vi "Ex seqlist.vi"() -> (0 "S array":T1(array[cluster]), 2 "selected Seq":string[](array[string]), 3 "selected sample name":string[](array[string]))   [LabVIEW 2018]
panel:
  in  "path":string="005.csv"
  in  "Select Base list":bool
  in  "All_Select":bool
  in  "Seqlist Renew":bool
  in  "Save":bool
  in  "load":bool
  out "size(s)":i32
  in  "Cluster":T2={"Right Read MIN"=6, "STD Type"=enum."Region", "Selection"=enum."10kHz", "Filter P"=0, "noise MAX"=3}
  out "S New Info and MiN out":T3={"Sample Sequence"="GATGATGATGATGATGAT", "Right Read MIN"=6, "Filter P"=0, "STD Type"=enum."Region", "Base Table"=[], "Selection"=enum."10kHz", "noise MAX"=3, "Sample name"=""} {"Base Table"."Value 3" format="%.2g"}
  out "Base Table":T4(array[cluster]) {"Value 3" format="%.2g"}
  out "Seq":string[](array[string])
  in  "EX":string[](array[string])
  out "All Ready?":bool
  in  "All_Clear":bool
  in  "Delete":bool
  out "F_Array":cluster{string, bool}[](array[cluster])
  out "Ready!":bool
  out "sorted array":string[](array[string])
  out "path 2":path
  out "SX#":i32
  out "location":string
  out "PC":string
  out "sample name":string[](array[string])
  in  "Go Net":bool
  in  "Scrollbar V 2":i32(c297)
  out "error out":errorcluster
  in  "error in":errorcluster
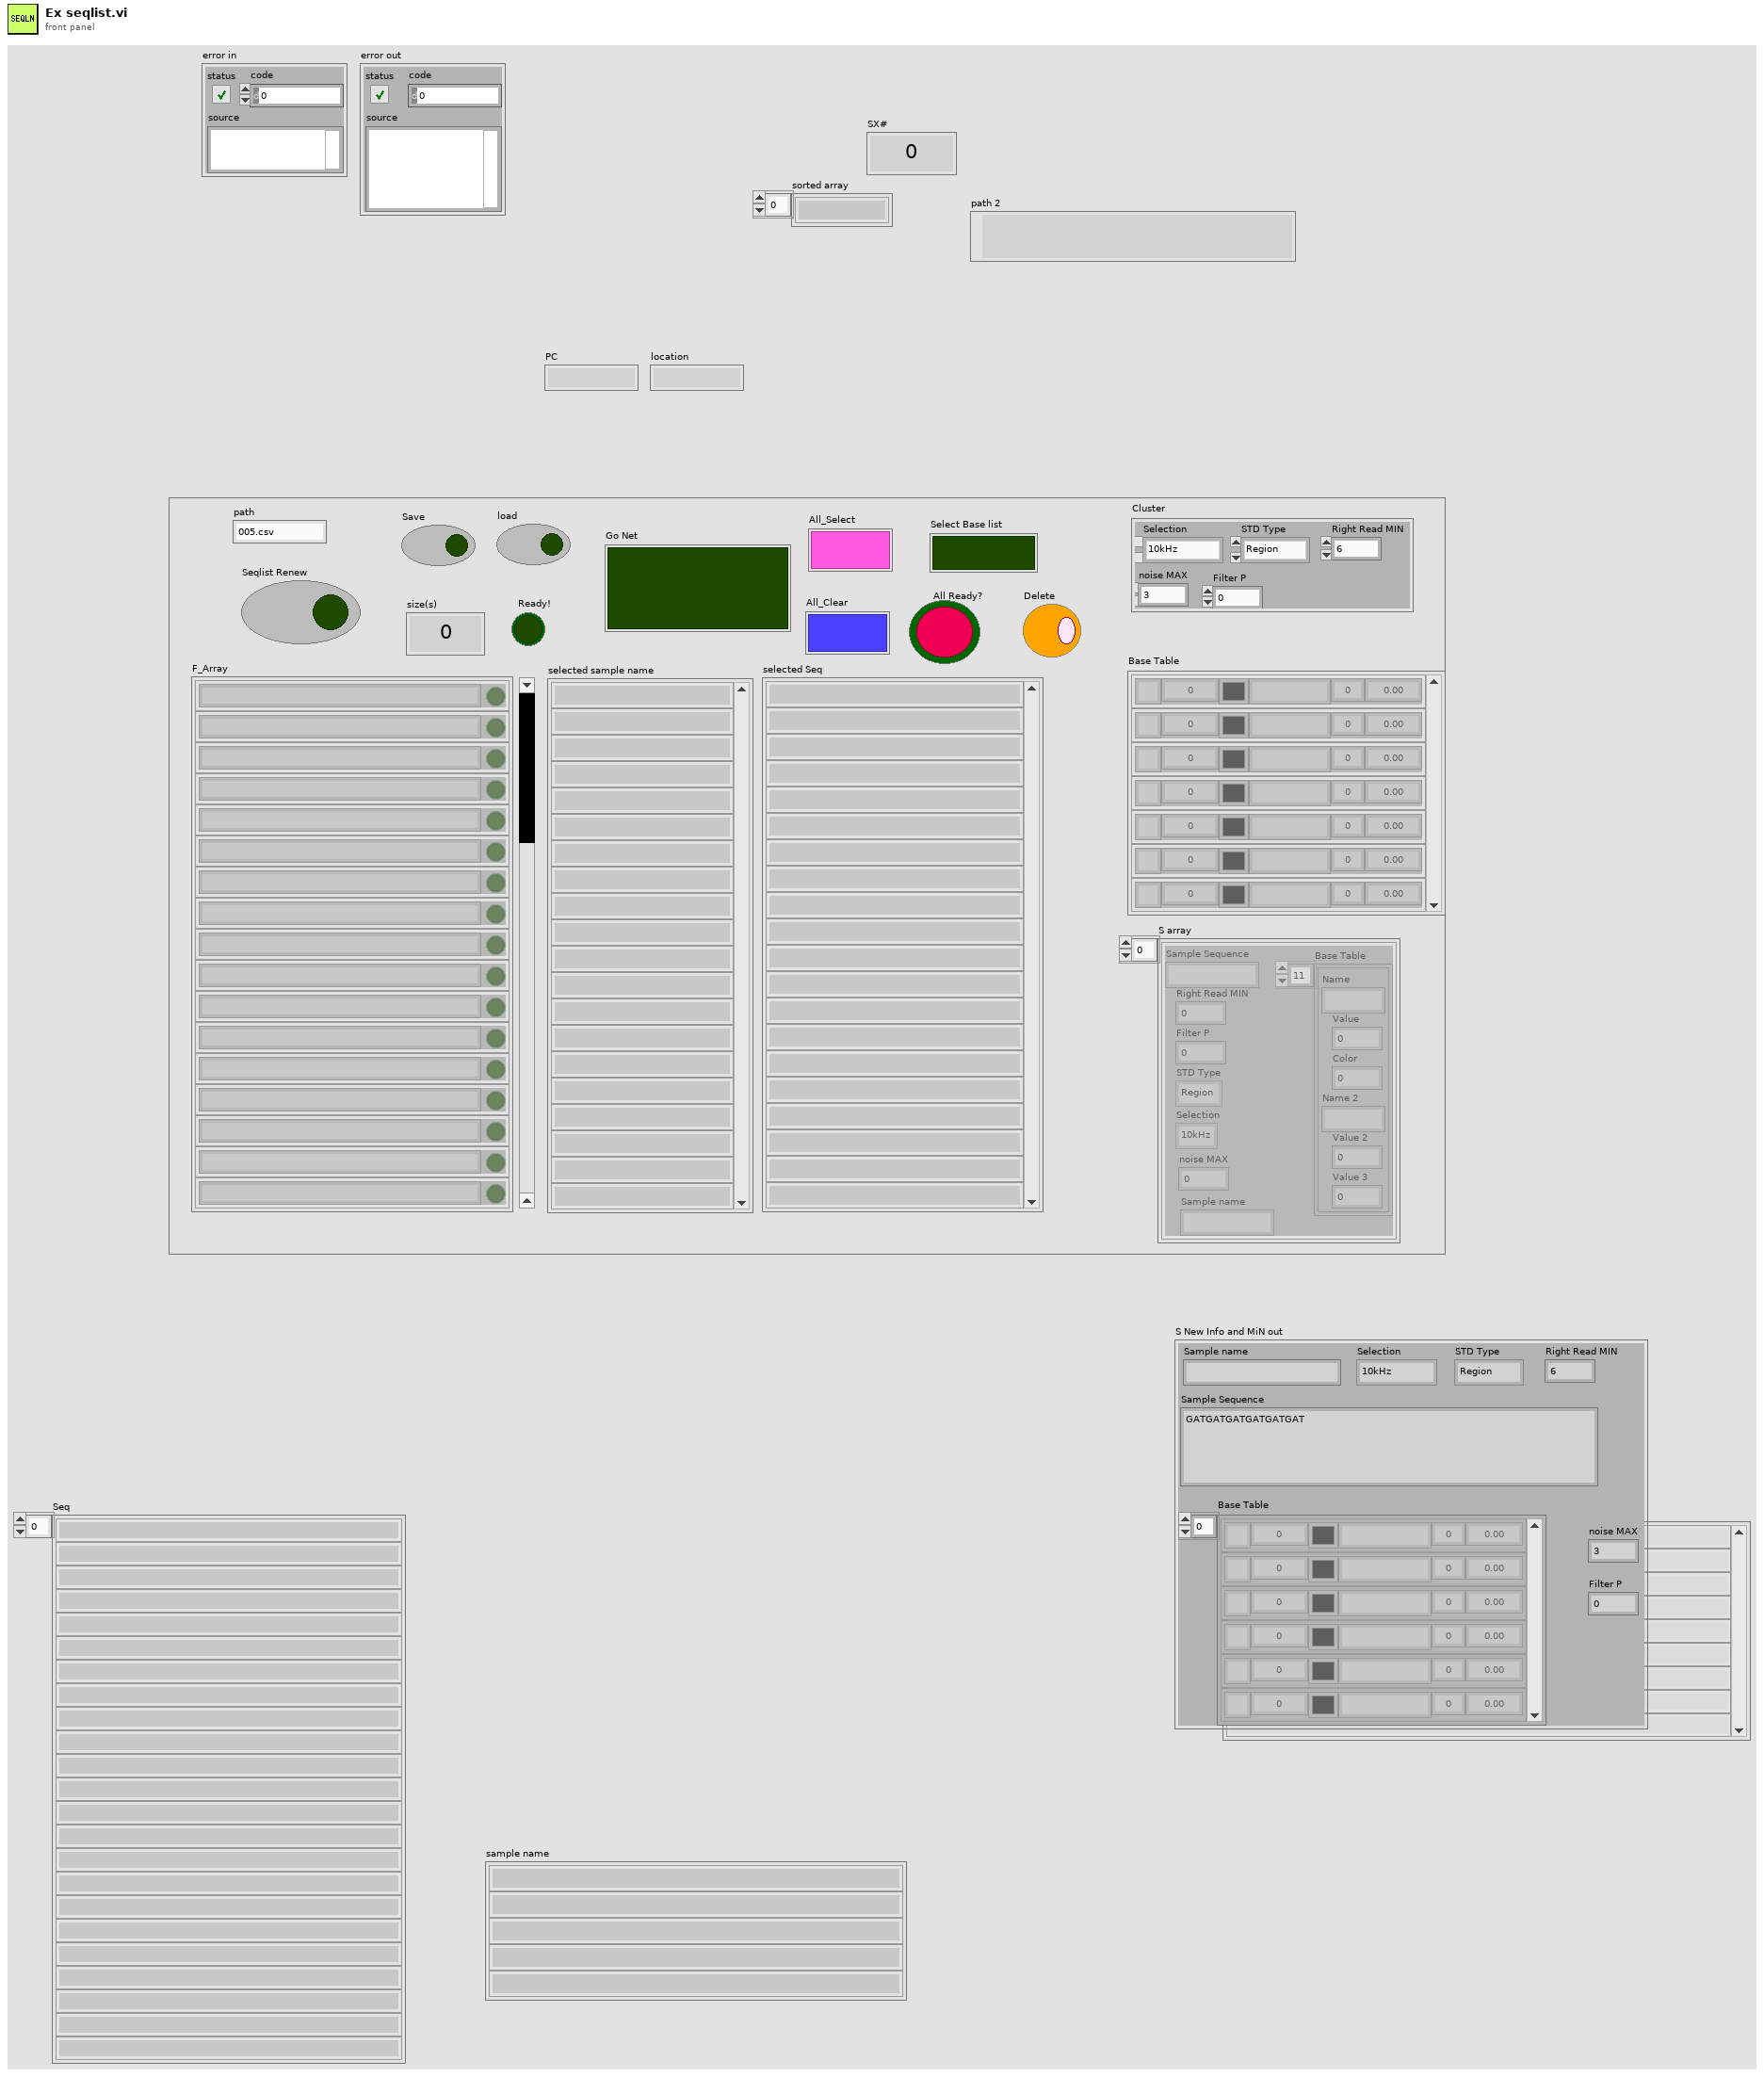
[diagram p1: front panel]
types:
  T1 = cluster{"Sample Sequence":string, "Right Read MIN":i32, "Filter P":i32, "STD Type":enum16{"Region", "Each", "Fixed"}, "Base Table":cluster{"Name":string, "Value":dbl, "Color":u32, "Name 2":string, "Value 2":dbl, "Value 3":dbl}[], "Selection":enum16{"10kHz", "100kHz"}, "noise MAX":i32, "Sample name":string}[]
  T2 = cluster{"Right Read MIN":i32, "STD Type":enum16{"Region", "Each", "Fixed"}, "Selection":enum16{"10kHz", "100kHz"}, "Filter P":i32, "noise MAX":i32}
  T3 = cluster{"Sample Sequence":string, "Right Read MIN":i32, "Filter P":i32, "STD Type":enum16{"Region", "Each", "Fixed"}, "Base Table":cluster{"Name":string, "Value":dbl, "Color":u32, "Name 2":string, "Value 2":dbl, "Value 3":dbl}[], "Selection":enum16{"10kHz", "100kHz"}, "noise MAX":i32, "Sample name":string}
  T4 = cluster{"Name":string, "Value":dbl, "Color":u32, "Name 2":string, "Value 2":dbl, "Value 3":dbl}[]
  T5 = cluster{"Sample ID":string, "Right Read MIN":i32, "Filter P":i32, "STD Type":enum16{"Region", "Each", "Fixed"}, "Base All Composition":cluster{"Name":string, "Value":dbl, "Color":u32, "Name 2":string, "Value 2":dbl, "Value 3":dbl}[], "Selection":enum16{"10kHz", "100kHz"}, "noise MAX":i32, string}[]
  T6 = typedef "LVPoint32TypeDef.ctl" = cluster{"Horizontal":i32, "Vertical":i32}
  T7 = typedef "LVPositionTypeDef.ctl" = cluster{"Left":i32, "Top":i32}
  T8 = typedef "LVBoundsTypeDef.ctl" = cluster{"Width":u32, "Height":u32}
  T9 = cluster{"Sample ID":string, "Right Read MIN":i32, "Filter P":i32, "STD Type":enum16{"Region", "Each", "Fixed"}, "Base All Composition":cluster{"Name":string, "Value":dbl, "Color":u32, "Name 2":string, "Value 2":dbl, "Value 3":dbl}[], "Selection":enum16{"10kHz", "100kHz"}, "noise MAX":i32, string}
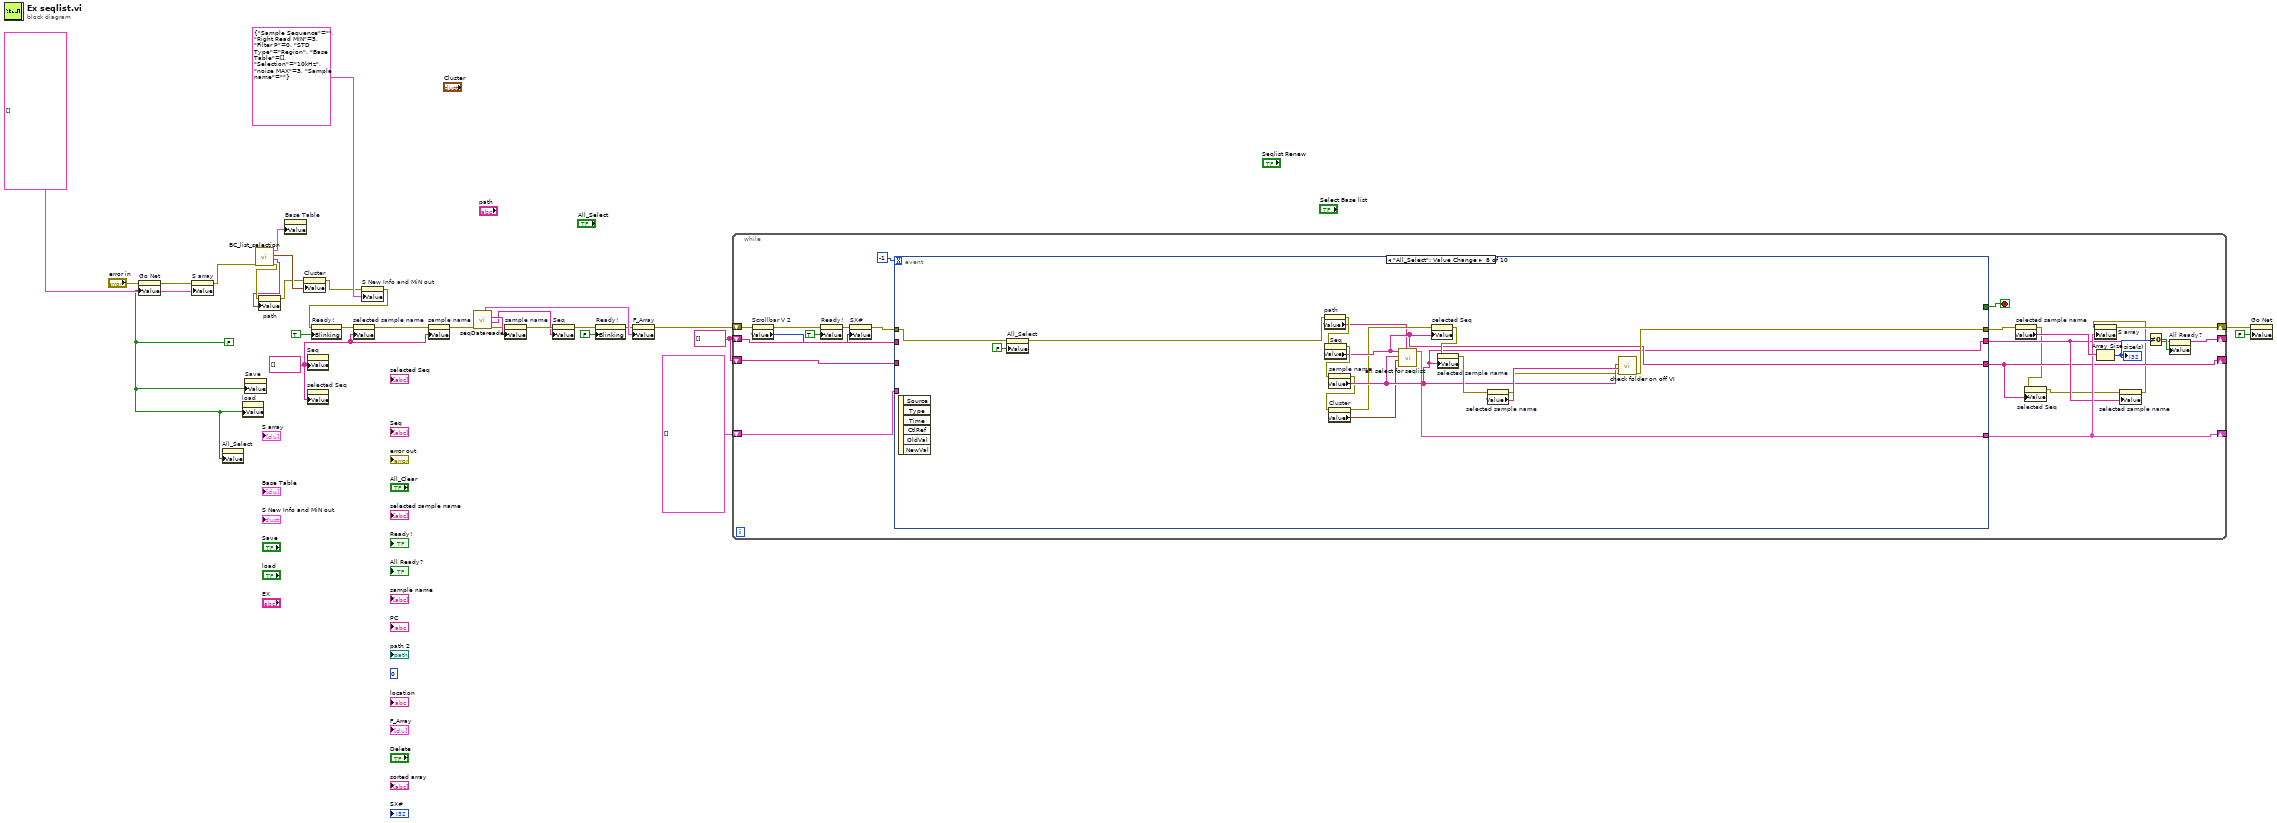
[diagram p0: block diagram]
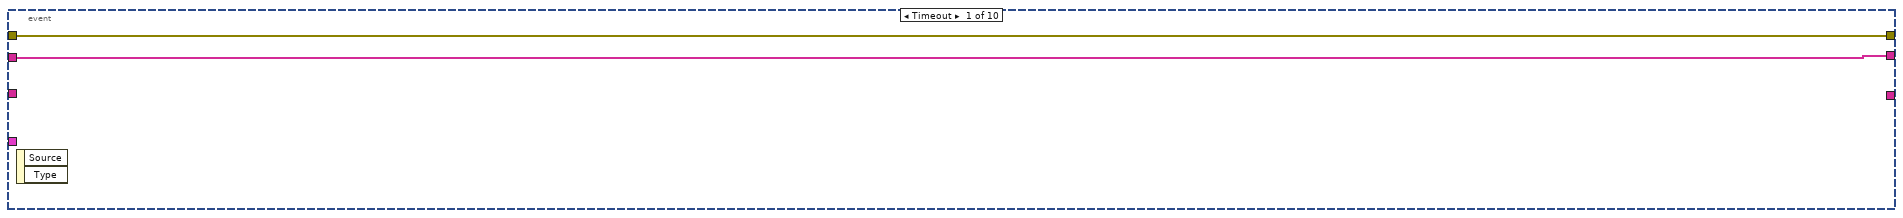
[diagram p2: hidden frame]
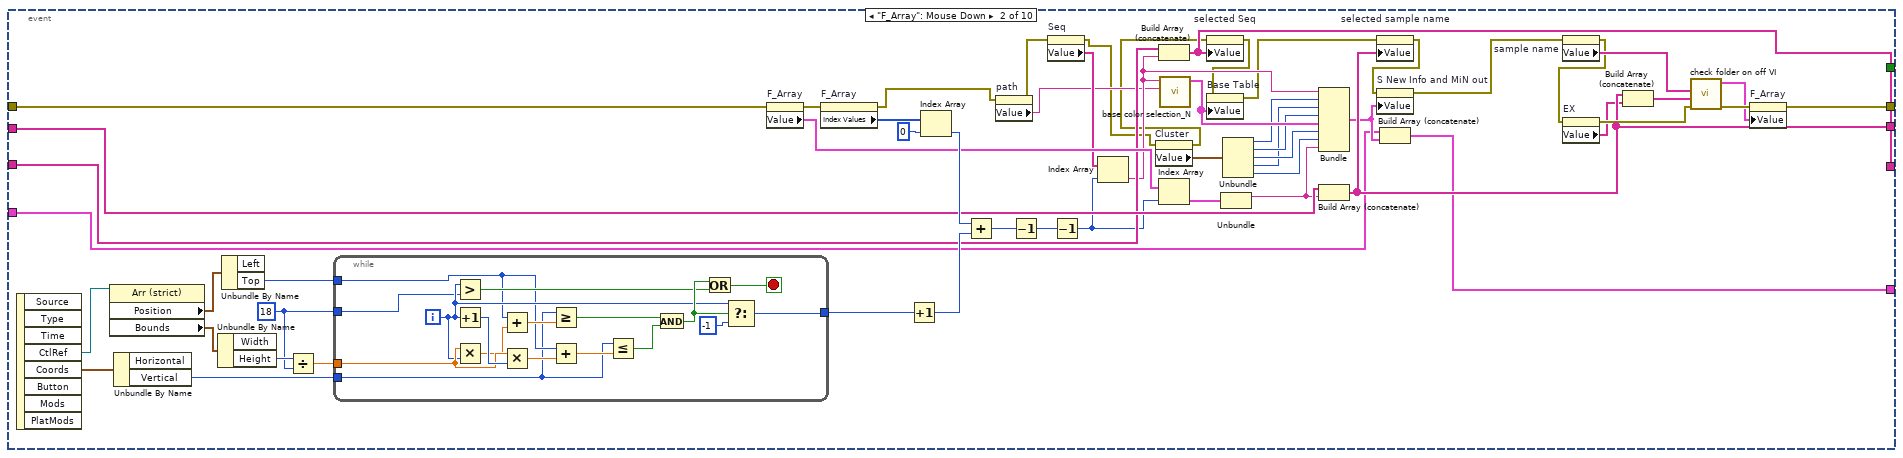
[diagram p3: hidden frame]
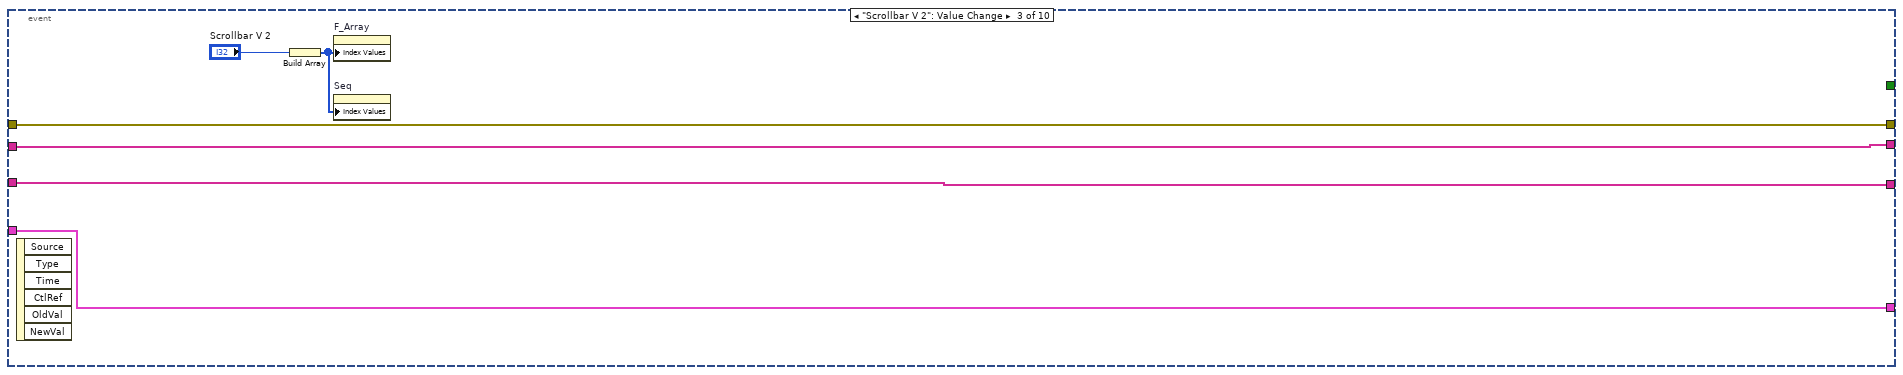
[diagram p4: hidden frame]
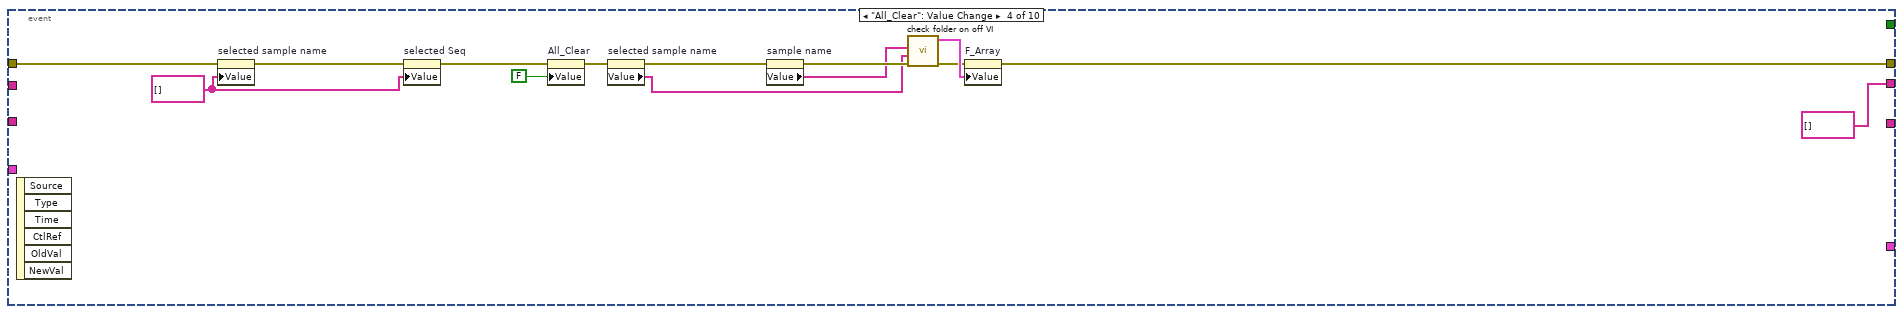
[diagram p5: hidden frame]
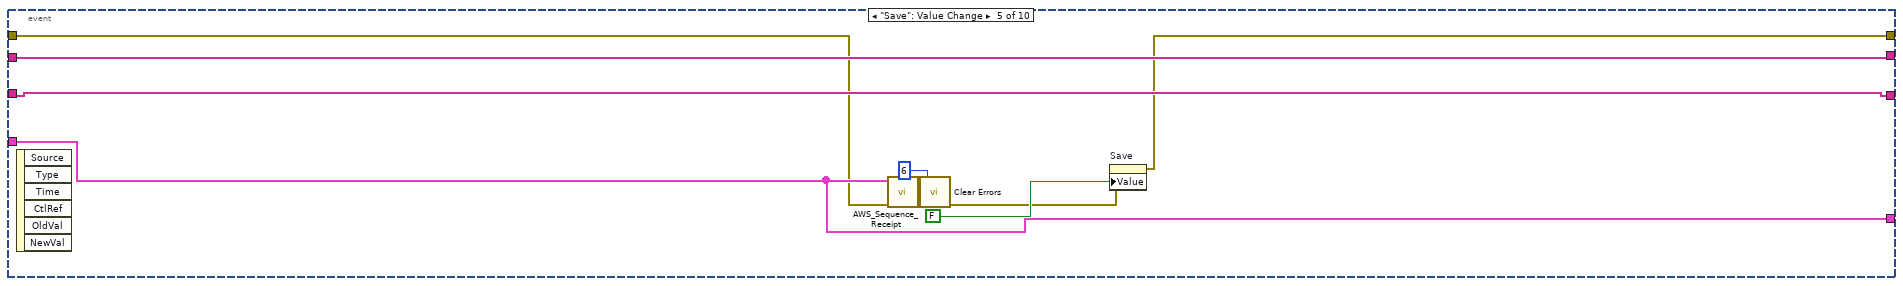
[diagram p6: hidden frame]
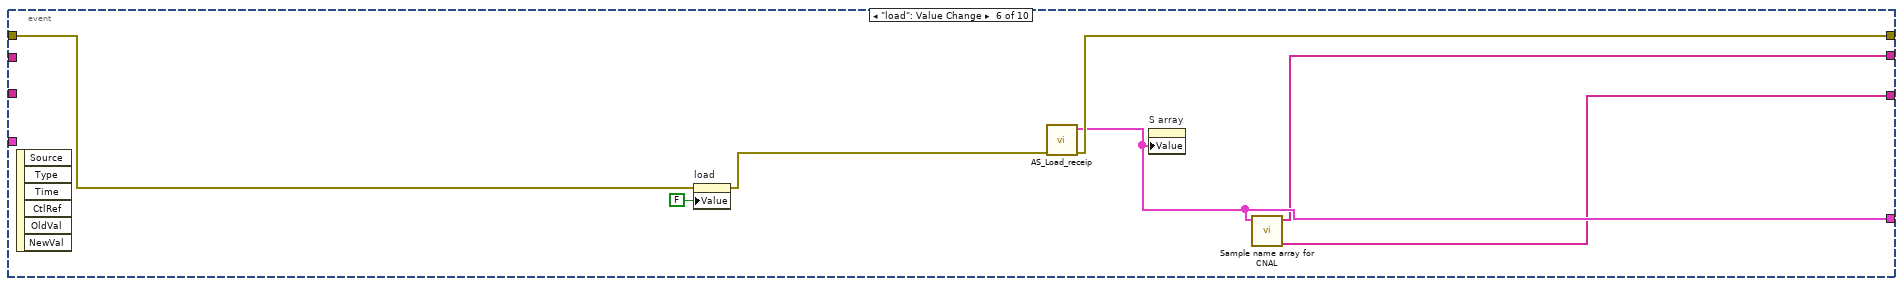
[diagram p7: hidden frame]
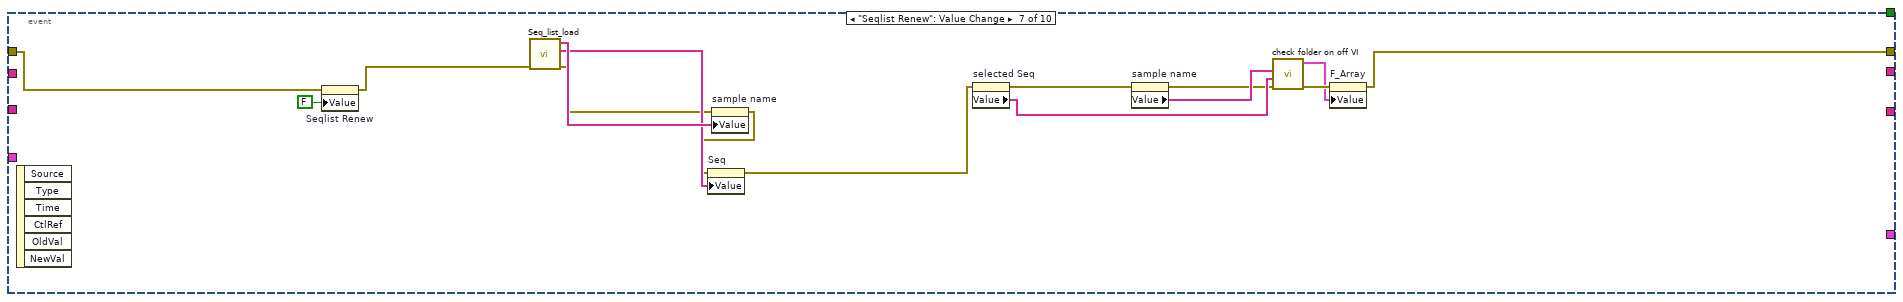
[diagram p8: hidden frame]
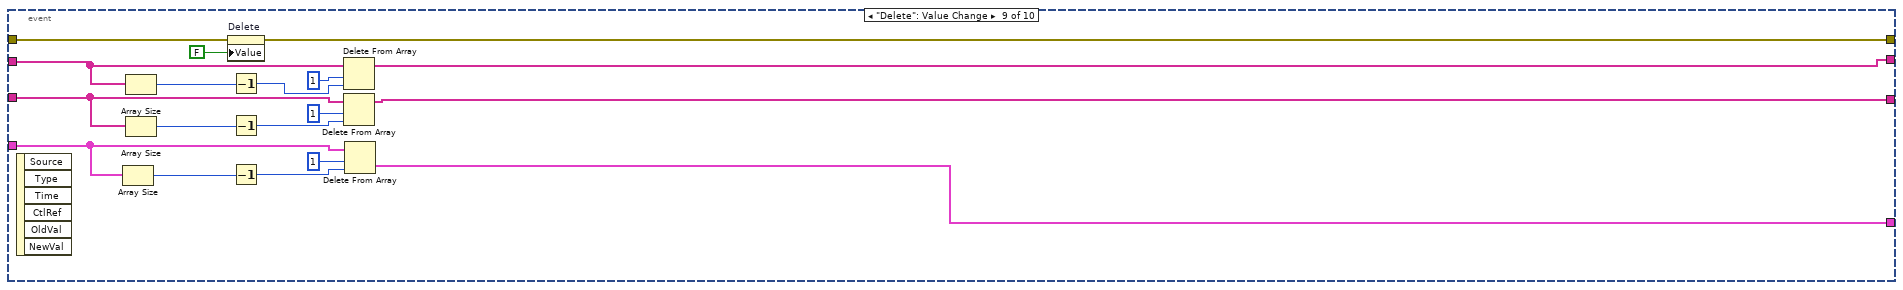
[diagram p9: hidden frame]
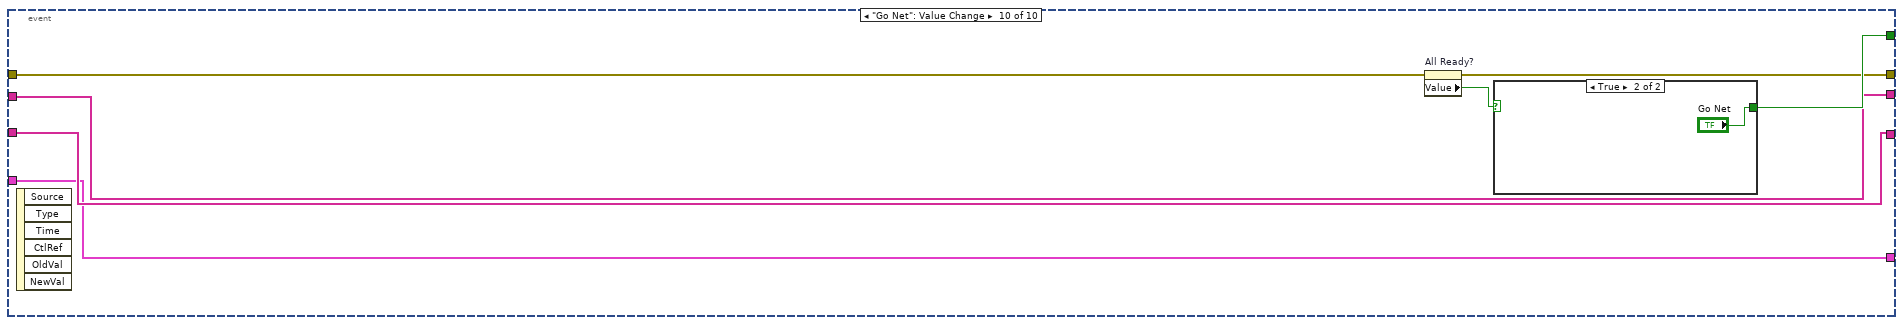
[diagram p10: hidden frame]
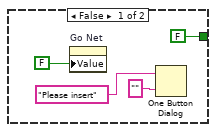
[diagram p11: hidden frame]
diagram:
  (unwired) 0 ("EX_IDX")
  w15 = string[] []
  w16 = string[] []
  w8 = FALSE ("10kHz_upload")
  n1 = property on="Go Net" class="Bool (strict)"(error in="error in", "Value"=w8) -> (error out=w11:errorcluster)  [unwired: 1 in, 1 out]
  n2 = property on="S array" class="Arr (strict)"(error in=w11, "Value"=T1 [] ("S array 2")) -> (error out=w5:errorcluster)  [unwired: 1 in, 1 out]
  n3 = property on="All_Select" class="Bool (strict)"("Value"=w8) -> ()  [unwired: 2 in, 2 out]
  n4 = property on="load" class="Bool (strict)"("Value"=w8) -> ()  [unwired: 2 in, 2 out]
  n5 = property on="Save" class="Bool (strict)"("Value"=w8) -> ()  [unwired: 2 in, 2 out]
  n6 = call "BC_list_selection.vi"("error in"=w5) -> ("error out"=w4:errorcluster, "path"=w2:string, "Cluster"=w6:T2, "Base All Composition"=w1:T4)  [unwired: 7 in]
  n7 = property on="path" class="Str"(error in=w4, "Value"=w2) -> (error out=w3:errorcluster)  [unwired: 1 in, 1 out]
  n8 = property on="Base Table" class="Arr (strict)"("Value"=w1) -> ()  [unwired: 2 in, 2 out]
  n9 = property on="Cluster" class="Clust (strict)"(error in=w3, "Value"=w6) -> (error out=w7:errorcluster)  [unwired: 1 in, 1 out]
  n10 = property on="Seq" class="Arr (strict)"("Value"=w15) -> ()  [unwired: 2 in, 2 out]
  n11 = property on="selected Seq" class="Arr (strict)"("Value"=w15) -> ()  [unwired: 2 in, 2 out]
  n12 = property on="S New Info and MiN out" class="Clust (strict)"(error in=w7, "Value"=T3 {"Sample Sequence"="", "Right Read MIN"=5, "Filter P"=0, "STD Type"=enum."Region", "Base Table"=[], "Selection"=enum."10kHz", "noise MAX"=3, "Sample name"=""} ("S New Info and MiN out 2")) -> (error out=w9:errorcluster)  [unwired: 1 in, 1 out]
  n13 = property on="Ready!" class="Bool (strict)"(error in=w9, "Blinking"=TRUE) -> (error out=w25:errorcluster)  [unwired: 1 in, 1 out]
  n14 = property on="selected sample name" class="Arr (strict)"(error in=w25, "Value"=w15) -> (error out=w27:errorcluster)  [unwired: 1 in, 1 out]
  n15 = property on="sample name" class="Arr (strict)"(error in=w27, "Value"=w15) -> (error out=w13:errorcluster)  [unwired: 1 in, 1 out]
  n16 = call "seqDatareader.vi"("エラー入力"=w13) -> ("error out"=w21:errorcluster, "Seq"=w17:string[], "Seq_name"=w22:string[], "Array 3"=w24:cluster{string, bool}[])  [unwired: 6 in, 1 out]
  n17 = property on="sample name" class="Arr (strict)"(error in=w21, "Value"=w22) -> (error out=w19:errorcluster)  [unwired: 1 in, 1 out]
  n18 = property on="Seq" class="Arr (strict)"(error in=w19, "Value"=w17) -> (error out=w18:errorcluster)  [unwired: 1 in, 1 out]
  n19 = property on="Ready!" class="Bool (strict)"(error in=w18, "Blinking"=FALSE ("Ready!")) -> (error out=w23:errorcluster)  [unwired: 1 in, 1 out]
  n20 = property on="F_Array" class="Arr (strict)"(error in=w23, "Value"=w24) -> (error out=w28:errorcluster)  [unwired: 1 in, 1 out]
  n21 = while {
    shift-right: [w36] -> _
    shift-left: w16 -> [w51]
    shift-right: [w37] -> w20
    shift-left: w28 -> [w50]
    shift-right: [w35] -> _
    shift-left: w16 -> [w41]
    shift-right: [w39] -> _
    shift-left: T5 [] -> [w40]
    stop <- w52 stop-if-true
    n22 = property on="Scrollbar V 2" class="Scroll (strict)"(error in=w50) -> (error out=w47:errorcluster, "Value"=w49:i32)  [unwired: 1 in, 1 out]
    n23 = property on="Ready!" class="Bool (strict)"(error in=w47, "Value"=TRUE ("Ready!")) -> (error out=w46:errorcluster)  [unwired: 1 in, 1 out]
    n24 = property on="SX#" class="DigNum (strict)"(error in=w46, "Value"=w49) -> (error out=w42:errorcluster)  [unwired: 1 in, 1 out]
    n25 = event shown="[7] \"All_Select\": Value Change" {
      selector: _ -> [_ _ _ _ _ _ _ _ _ _]
      dyn-events: _ -> [_ _ _ _ _ _ _ _ _ _]
      timeout: -1 -> [_ _ _ _ _ _ _ _ _ _]
      tunnel: [w55 w89 w132 w140 w148 w163 w164 w191 w211 w217] -> w44
      tunnel: [w54 w85 w133 string[] [] w151 w161 _ w186 w200 w219] -> w36
      tunnel: w51 -> [w54 w92 w133 _ w151 _ _ _ w198 w219]
      tunnel: [_ _ _ _ _ _ _ _ _ w220] -> w52
      tunnel: w42 -> [w55 w82 w132 w139 w149 w158 w177 w195 w212 w218]
      tunnel: w41 -> [_ w81 w129 _ w150 _ _ _ w196 w215]
      tunnel: [_ w78 w129 _ w150 w160 _ w187 w199 w215] -> w35
      tunnel: [_ w66 w128 _ w152 w162 _ w192 w201 w214] -> w39
      tunnel: w40 -> [_ w67 w128 _ w152 _ _ _ w197 w214]
      event Timeout {
        n26 = event-data() -> ()  [unwired: 1 in, 2 out]
      }
      event "F_Array": Mouse Down {
        w102 = 18 ("f")
        n27 = event-data() -> ("CtlRef"=w94:refnum<vi>, "Coords"=w93:T6)  [unwired: 1 in, 6 out]
        n28 = property class="Arr (strict)"(reference=w94) -> ("Position"=w108:T7, "Bounds"=w107:T8)  [unwired: 1 in, 2 out]
        n29 = Unbundle By Name(w93) -> ("Vertical"=w106:i32)  [unwired: 1 out]
        n30 = Unbundle By Name(w107) -> ("Height"=w105:u32)  [unwired: 1 out]
        n31 = Unbundle By Name(w108) -> ("Top"=w103:i32)  [unwired: 1 out]
        n32 = Divide(x=w105, y=w102) -> (x/y=w104:dbl)
        n33 = while {
          tunnel: w106 -> [w111]
          tunnel: w104 -> [w117]
          tunnel: w103 -> [w113]
          tunnel: [w122] -> w98
          tunnel: w102 -> [w112]
          i -> [w116]
          stop <- w120 stop-if-true
          n34 = Greater?(x=w116, y=w112) -> (0:w118:bool)
          n35 = Increment(x=w116) -> (x+1=w127:i32)
          n36 = Multiply(x=w117, y=w116) -> (x*y=w114:dbl)
          n37 = Add(x=w113, y=w114) -> (x+y=w115:dbl)
          n38 = Multiply(x=w117, y=w127) -> (x*y=w125:dbl)
          n39 = Greater Or Equal?(x=w111, y=w115) -> (x >= y?=w124:bool)
          n40 = Add(x=w113, y=w125) -> (x+y=w126:dbl)
          n41 = Less Or Equal?(x=w111, y=w126) -> (x <= y?=w123:bool)
          n42 = And(x=w124, y=w123) -> (x .and. y?=w119:bool)
          n43 = Or(x=w119, y=w118) -> (x .or. y?=w120:bool)
          n44 = Select(t=w116, s=w119, f=-1) -> (s? t:f=w122:i32)
        }
        n45 = property on="F_Array" class="Arr (strict)"(error in=w82) -> (error out=w96:errorcluster, "Value"=w97:cluster{string, bool}[])  [unwired: 1 in, 1 out]
        n46 = property on="F_Array" class="Arr (strict)"(error in=w96) -> (error out=w62:errorcluster, "Index Values"=w109:u32[])  [unwired: 1 in, 1 out]
        n47 = Increment(x=w98) -> (x+1=w101:i32)
        n48 = Index Array(array=w109, index=0 ("指標")) -> (element=w99:u32)
        n49 = Add(x=w99, y=w101) -> (x+y=w100:u32)
        n50 = property on="path" class="Str"(error in=w62) -> (error out=w61:errorcluster, "Value"=w65:string)  [unwired: 1 in, 1 out]
        n51 = Decrement(x=w100) -> (x-1=w95:u32)
        n52 = property on="Seq" class="Arr (strict)"(error in=w61) -> (error out=w64:errorcluster, "Value"=w80:string[])  [unwired: 1 in, 1 out]
        n53 = Decrement(x=w95) -> (x-1=w79:u32)
        n54 = Index Array(array=w80, index=w79) -> (element=w75:string)
        n55 = property on="Cluster" class="Clust (strict)"(error in=w64) -> (error out=w63:errorcluster, "Value"=w74:T2)  [unwired: 1 in, 1 out]
        n56 = Build Array (concatenate)(w81, w75) -> (w78:string[])
        n57 = Index Array(array=w97, index=w79) -> (element=w91:cluster{string, bool})
        n58 = call "base color selection_N.vi"("path"=w65, "Sample Sequence"=w75) -> ("Base All Composition"=w77:T4)  [unwired: 8 in, 1 out]
        n59 = property on="selected Seq" class="Arr (strict)"(error in=w63, "Value"=w78) -> (error out=w60:errorcluster)  [unwired: 1 in, 1 out]
        n60 = property on="Base Table" class="Arr (strict)"(error in=w60, "Value"=w77) -> (error out=w59:errorcluster)  [unwired: 1 in, 1 out]
        n61 = Unbundle(w91) -> (w76:string)  [unwired: 1 out]
        n62 = Unbundle(w74) -> ("Right Read MIN"=w73:i32, "STD Type"=w72:enum16{"Region", "Each", "Fixed"}, "Selection"=w71:enum16{"10kHz", "100kHz"}, "Filter P"=w69:i32, "noise MAX"=w70:i32)
        n63 = Bundle("Sample ID"=w75, "Right Read MIN"=w73, "Filter P"=w69, "STD Type"=w72, "Base All Composition"=w77, "Selection"=w71, "noise MAX"=w70, w76) -> (w68:T9)  [unwired: 1 in]
        n64 = Build Array (concatenate)(w92, w76) -> (w85:string[])
        n65 = property on="selected sample name" class="Arr (strict)"(error in=w59, "Value"=w85) -> (error out=w58:errorcluster)  [unwired: 1 in, 1 out]
        n66 = property on="S New Info and MiN out" class="Clust (strict)"(error in=w58, "Value"=w68) -> (error out=w57:errorcluster)  [unwired: 1 in, 1 out]
        n67 = Build Array (concatenate)(w67, w68) -> (w66:T5)
        n68 = property on="sample name" class="Arr (strict)"(error in=w57) -> (error out=w56:errorcluster, "Value"=w86:string[])  [unwired: 1 in, 1 out]
        n69 = property on="EX" class="Arr (strict)"(error in=w56) -> (error out=w87:errorcluster, "Value"=w84:string[])  [unwired: 1 in, 1 out]
        n70 = Build Array (concatenate)(w85, w84) -> (w83:string[])
        n71 = call "check folder on off VI.vi"("エラー入力"=w87, "selected EX"=w83, "folder names"=w86) -> ("error out"=w90:errorcluster, "Array 3"=w88:cluster{string, bool}[])  [unwired: 6 in, 1 out]
        n72 = property on="F_Array" class="Arr (strict)"(error in=w90, "Value"=w88) -> (error out=w89:errorcluster)  [unwired: 1 in, 1 out]
      }
      event "Scrollbar V 2": Value Change {
        n73 = event-data() -> ()  [unwired: 1 in, 6 out]
        n74 = Build Array("Scrollbar V 2") -> (w130:i32[])
        n75 = property on="F_Array" class="Arr (strict)"("Index Values"=w130) -> ()  [unwired: 2 in, 2 out]
        n76 = property on="Seq" class="Arr (strict)"("Index Values"=w130) -> ()  [unwired: 2 in, 2 out]
      }
      event "All_Clear": Value Change {
        w136 = string[] []
        n77 = event-data() -> ()  [unwired: 1 in, 6 out]
        n78 = property on="selected sample name" class="Arr (strict)"(error in=w139, "Value"=w136) -> (error out=w135:errorcluster)  [unwired: 1 in, 1 out]
        n79 = property on="selected Seq" class="Arr (strict)"(error in=w135, "Value"=w136) -> (error out=w134:errorcluster)  [unwired: 1 in, 1 out]
        n80 = property on="All_Clear" class="Bool (strict)"(error in=w134, "Value"=FALSE ("All_Clear")) -> (error out=w138:errorcluster)  [unwired: 1 in, 1 out]
        n81 = property on="selected sample name" class="Arr (strict)"(error in=w138) -> (error out=w137:errorcluster, "Value"=w143:string[])  [unwired: 1 in, 1 out]
        n82 = property on="sample name" class="Arr (strict)"(error in=w137) -> (error out=w145:errorcluster, "Value"=w144:string[])  [unwired: 1 in, 1 out]
        n83 = call "check folder on off VI.vi"("エラー入力"=w145, "selected EX"=w143, "folder names"=w144) -> ("error out"=w141:errorcluster, "Array 3"=w142:cluster{string, bool}[])  [unwired: 6 in, 1 out]
        n84 = property on="F_Array" class="Arr (strict)"(error in=w141, "Value"=w142) -> (error out=w140:errorcluster)  [unwired: 1 in, 1 out]
      }
      event "Save": Value Change {
        n85 = event-data() -> ()  [unwired: 1 in, 6 out]
        n86 = call "AWS_Sequence_Receipt.vi"("error in"=w149, "S array"=w152) -> ("error out"=w156:errorcluster)  [unwired: 7 in, 2 out]
        n87 = call <vilib>:"Clear Errors.vi"("error in (no error)"=w156, "specific error code to clear (0: all)"=6) -> ("error out"=w154:errorcluster)  [unwired: 4 in, 1 out]
        n88 = property on="Save" class="Bool (strict)"(error in=w154, "Value"=FALSE ("Save")) -> (error out=w148:errorcluster)  [unwired: 1 in, 1 out]
      }
      event "load": Value Change {
        n89 = event-data() -> ()  [unwired: 1 in, 6 out]
        n90 = property on="load" class="Bool (strict)"(error in=w158, "Value"=FALSE ("load")) -> (error out=w157:errorcluster)  [unwired: 1 in, 1 out]
        n91 = call "AS_Load_receip.vi"("error in"=w157) -> ("error out"=w163:errorcluster, "S array"=w162:T1)  [unwired: 9 in]
        n92 = property on="S array" class="Arr (strict)"("Value"=w162) -> ()  [unwired: 2 in, 2 out]
        n93 = call "Sample name array for CNAL.vi"("S array"=w162) -> ("Sample Sequence array"=w160:string[], "Sample name array"=w161:string[])  [unwired: 9 in]
      }
      event "Seqlist Renew": Value Change {
        n94 = event-data() -> ()  [unwired: 1 in, 6 out]
        n95 = property on="Seqlist Renew" class="Bool (strict)"(error in=w177, "Value"=FALSE ("Seqlist Renew")) -> (error out=w176:errorcluster)  [unwired: 1 in, 1 out]
        n96 = call "Seq_list_load.vi"("error in"=w176) -> ("error out"=w167:errorcluster, "selected Seq"=w168:string[], "selected sample name"=w169:string[])  [unwired: 8 in]
        n97 = property on="sample name" class="Arr (strict)"(error in=w167, "Value"=w169) -> (error out=w166:errorcluster)  [unwired: 1 in, 1 out]
        n98 = property on="Seq" class="Arr (strict)"(error in=w166, "Value"=w168) -> (error out=w165:errorcluster)  [unwired: 1 in, 1 out]
        n99 = property on="selected Seq" class="Arr (strict)"(error in=w165) -> (error out=w175:errorcluster, "Value"=w172:string[])  [unwired: 1 in, 1 out]
        n100 = property on="sample name" class="Arr (strict)"(error in=w175) -> (error out=w170:errorcluster, "Value"=w171:string[])  [unwired: 1 in, 1 out]
        n101 = call "check folder on off VI.vi"("エラー入力"=w170, "selected EX"=w172, "folder names"=w171) -> ("error out"=w174:errorcluster, "Array 3"=w173:cluster{string, bool}[])  [unwired: 6 in, 1 out]
        n102 = property on="F_Array" class="Arr (strict)"(error in=w174, "Value"=w173) -> (error out=w164:errorcluster)  [unwired: 1 in, 1 out]
      }
      event "All_Select": Value Change {
        n103 = event-data() -> ()  [unwired: 1 in, 6 out]
        n104 = property on="All_Select" class="Bool (strict)"(error in=w195, "Value"=FALSE ("All_Select")) -> (error out=w181:errorcluster)  [unwired: 1 in, 1 out]
        n105 = property on="path" class="Str"(error in=w181) -> (error out=w180:errorcluster, "Value"=w179:string)  [unwired: 1 in, 1 out]
        n106 = property on="Seq" class="Arr (strict)"(error in=w180) -> (error out=w193:errorcluster, "Value"=w187:string[])  [unwired: 1 in, 1 out]
        n107 = property on="sample name" class="Arr (strict)"(error in=w193) -> (error out=w184:errorcluster, "Value"=w186:string[])  [unwired: 1 in, 1 out]
        n108 = property on="Cluster" class="Clust (strict)"(error in=w184) -> (error out=w183:errorcluster, "Value"=w182:T2)  [unwired: 1 in, 1 out]
        n109 = call "all select for seqlist.vi"("path"=w179, "Cluster"=w182, "sample name"=w186, "Seq"=w187) -> ("S array"=w192:T1)  [unwired: 7 in]
        n110 = property on="selected Seq" class="Arr (strict)"(error in=w183, "Value"=w187) -> (error out=w189:errorcluster)  [unwired: 1 in, 1 out]
        n111 = property on="selected sample name" class="Arr (strict)"(error in=w189, "Value"=w186) -> (error out=w188:errorcluster)  [unwired: 1 in, 1 out]
        n112 = property on="selected sample name" class="Arr (strict)"(error in=w188) -> (error out=w185:errorcluster, "Value"=w190:string[])  [unwired: 1 in, 1 out]
        n113 = call "check folder on off VI.vi"("エラー入力"=w185, "selected EX"=w190, "folder names"=w186) -> ("error out"=w191:errorcluster)  [unwired: 6 in, 2 out]
      }
      event "Delete": Value Change {
        n114 = event-data() -> ()  [unwired: 1 in, 6 out]
        n115 = Array Size(array=w197) -> (size(s)=w203:i32)
        n116 = Array Size(array=w198) -> (size(s)=w206:i32)
        n117 = Array Size(array=w196) -> (size(s)=w209:i32)
        n118 = property on="Delete" class="Bool (strict)"(error in=w212, "Value"=FALSE ("DF_enter")) -> (error out=w211:errorcluster)  [unwired: 1 in, 1 out]
        n119 = Decrement(x=w206) -> (x-1=w205:i32)
        n120 = Decrement(x=w209) -> (x-1=w208:i32)
        n121 = Decrement(x=w203) -> (x-1=w202:i32)
        n122 = Delete From Array(array=w198, length=1 ("長さ"), index=w205) -> (array with subset deleted=w200:string[])  [unwired: 1 out]
        n123 = Delete From Array(array=w196, length=1 ("長さ"), index=w208) -> (array with subset deleted=w199:string[])  [unwired: 1 out]
        n124 = Delete From Array(array=w197, length=1 ("長さ"), index=w202) -> (deleted portion=w201:T5)  [unwired: 1 out]
      }
      event "Go Net": Value Change {
        n125 = event-data() -> ()  [unwired: 1 in, 6 out]
        n126 = property on="All Ready?" class="Bool (strict)"(error in=w218) -> (error out=w217:errorcluster, "Value"=w216:bool)  [unwired: 1 in, 1 out]
        n127 = case shown="True" w216 {
          tunnel: [FALSE ("END") "Go Net"] -> w220
          frame False {
            n128 = property on="Go Net" class="Bool (strict)"("Value"=FALSE ("All Ready?")) -> ()  [unwired: 2 in, 2 out]
            n129 = One Button Dialog(message="Please insert", button name ("OK")="") -> ()  [unwired: 1 out]
          }
          frame True {
          }
        }
      }
    }
    n130 = property on="selected sample name" class="Arr (strict)"(error in=w44) -> (error out=w34:errorcluster, "Value"=w45:string[])  [unwired: 1 in, 1 out]
    n131 = property on="selected Seq" class="Arr (strict)"(error in=w34, "Value"=w35) -> (error out=w33:errorcluster)  [unwired: 1 in, 1 out]
    n132 = Array Size(array=w45) -> (size(s)=w43:i32)
    "size(s)" <- w43
    n133 = property on="selected sample name" class="Arr (strict)"(error in=w33, "Value"=w36) -> (error out=w32:errorcluster)  [unwired: 1 in, 1 out]
    n134 = property on="S array" class="Arr (strict)"(error in=w32, "Value"=w39) -> (error out=w37:errorcluster)  [unwired: 1 in, 1 out]
    n135 = Not Equal To 0?(x=w43) -> (x != 0?=w38:bool)
    n136 = property on="All Ready?" class="Bool (strict)"("Value"=w38) -> ()  [unwired: 2 in, 2 out]
  }
  n137 = property on="Go Net" class="Bool (strict)"(error in=w20, "Value"=FALSE ("END")) -> ()  [unwired: 1 in, 2 out]
